vi "Read U64.vi"(8 "error in (no error)":errorcluster, 9 "Timeout (ms)":i32, 11 "CIFTag in":refnum<class "CIF_Iceoryx_Chn_U64.lvclass">) -> (0 "error out":errorcluster, 1 "timed out?":bool, 2 "Data":u64, 3 "CIFTag out":refnum<class "CIF_Iceoryx_Chn_U64.lvclass">)   [LabVIEW 2021, in "CIF_Iceoryx_Chn_U64.lvclass"]
uses:
  CIF_Iceoryx_Chn_U64.lvclass
  D:/dev/Packages/CIF_Channels_Core/src/CIFChannels/CIFChannels.lvclass
  D:/dev/Packages/CIF_Channels_Core/src/Iceorxy_Channels/CIF_Iceoryx_BB/CIF_Iceoryx_BB.lvclass
  CIFChannels/CIFChannels.lvclass/CIFChannels.ctl
  CIF_Iceoryx_Chn_U64.lvclass/CIF_Iceoryx_Chn_U64.ctl
  CIF_Iceoryx_BB/CIF_Iceoryx_BB.lvclass/CIF_Iceoryx_BB.ctl
  CIF_Iceoryx_BB/Accessors/Read Reader Reference.vi
  Read U64 Direct.vi/959f43c0-2965-45e0-a797-017a19813e3c.vi
  CIFChannels/Accessors/Read Channel State.vi
  CIFChannels/Accessors/Read Direction.vi
  CIFChannels/Accessors/Read Tag Forced.vi
  <vilib>/CIF Foundation/CIF Iceoryx/SubVIs/Get Path.vi
  <vilib>/CIF Foundation/CIF Iceoryx/SubVIs/Convert Error.vi
  <vilib>/CIF Foundation/CIF Iceoryx/Refnum/BB Reader from Refnum.vi
  <vilib>/CIF Foundation/CIF Iceoryx/SubVIs/Convert Error Core.vi
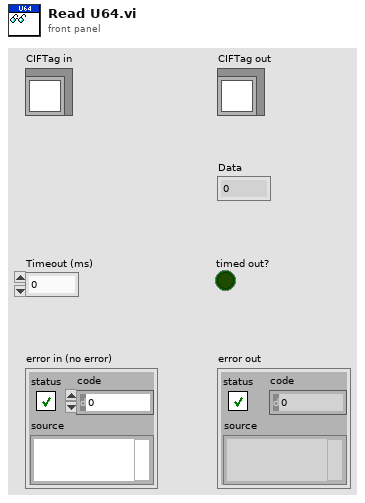
[diagram p1: front panel]
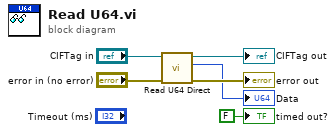
[diagram p0: block diagram]
diagram:
  n1 = call "Read U64 Direct.vi"("error in (no error)"="error in (no error)", "CIFTag in"="CIFTag in") -> ("error out"=→"error out":errorcluster, "Data"=→"Data":u64, "CIFTag out"=→"CIFTag out":refnum<class "CIF_Iceoryx_Chn_U64.lvclass">)  [unwired: 7 in]
  "timed out?" <- FALSE ("timed out?")
